vi "UMLEditor CreateNoteText.vi"(1 "graph":refnum<class "Graph.lvclass">, 2 "NoteEdge?":refnum<class "AbstractEdge.lvclass">, 5 "error in (no error)":errorcluster) -> (19 "error out":errorcluster)   [LabVIEW 2020]
doc: "Gets current diagram values"
uses:
  <resource>/Framework/Providers/Open_GDS/UML/Graph_class/Graph.lvclass
  <resource>/Framework/Providers/Open_GDS/UML/AbstractEdge_class/AbstractEdge.lvclass
  <resource>/Framework/Providers/Open_GDS/UML/General/Point/Point Point2D.ctl
  <resource>/Framework/Providers/Open_GDS/UML/NoteNode_class/NoteNode.lvclass
  <resource>/Framework/Providers/Open_GDS/UML/AbstractNode_class/AbstractNode.lvclass
  <resource>/Framework/Providers/Open_GDS/UML/MultiLineString_class/MultiLineString.lvclass
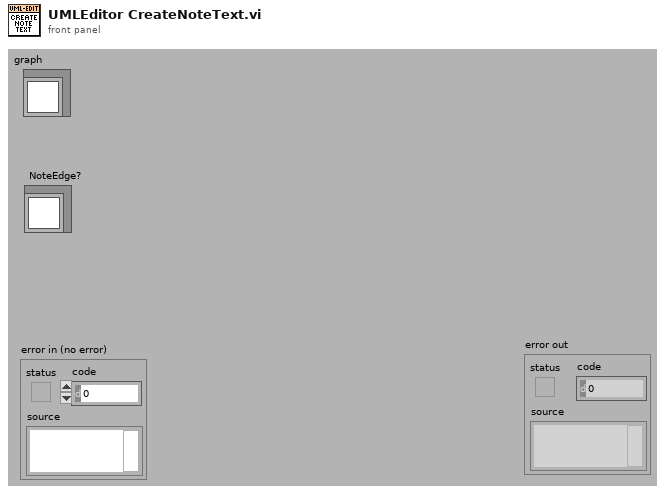
[diagram p1: front panel]
types:
  T1 = typedef "Point Point2D.ctl" = cluster{"x":dbl, "y":dbl}
  T2 = cluster{"text":string, "empty picture":picture, string}
  T3 = typedef "Rectangle Rectangle2D.ctl" = cluster{"x":dbl, "y":dbl, "width":dbl, "height":dbl}
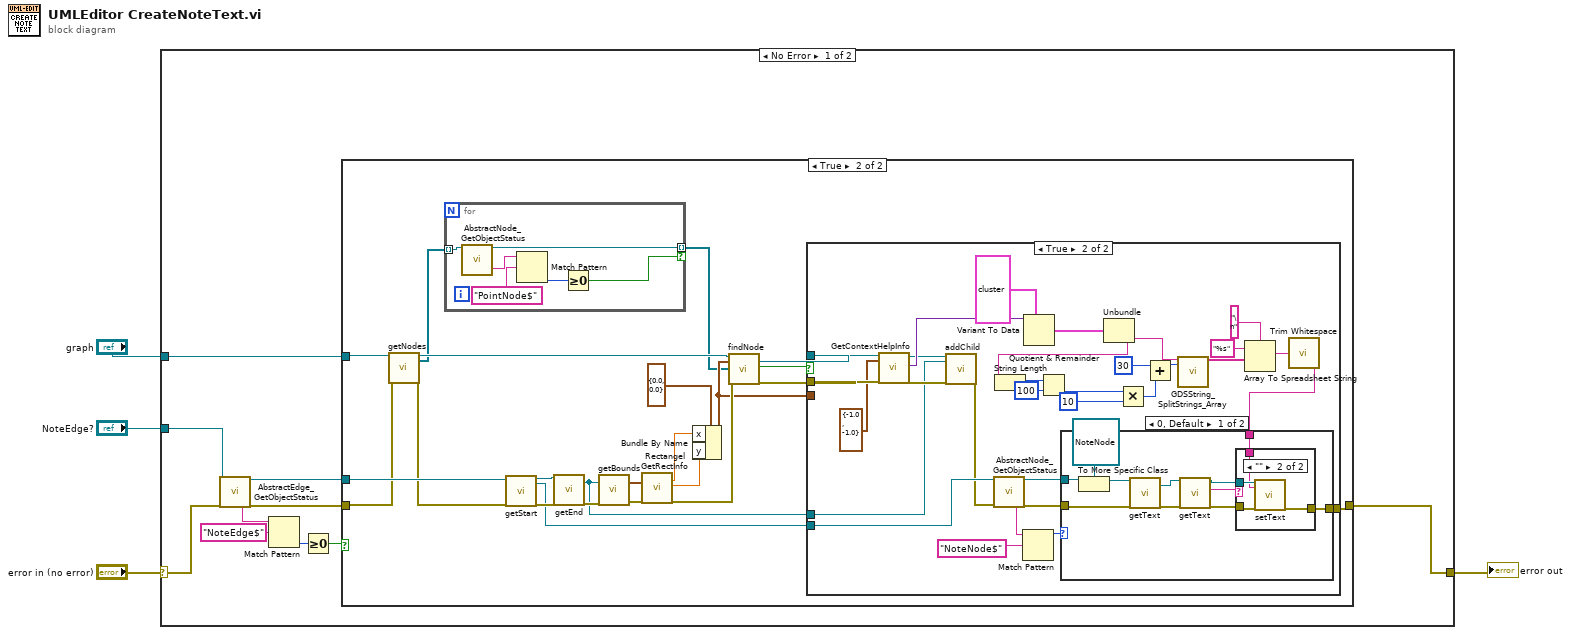
[diagram p0: block diagram]
diagram:
  n1 = case shown="No Error" "error in (no error)" {
    selector: "error in (no error)" -> [w8 w93]
    tunnel: [w7 w93] -> w3
    tunnel: "NoteEdge?" -> [w10 _]
    tunnel: "graph" -> [w6 _]
    frame No Error {
      n2 = call <resource>:"AbstractEdge_GetObjectStatus.vi"("reference in"=w10, "error in (no error)"=w8) -> ("Class name"=w13:string, "reference out"=w5:refnum<class "AbstractEdge.lvclass">, "error out"=w14:errorcluster)  [unwired: 9 in, 6 out]
      n3 = Match Pattern(string=w13, regular expression="NoteEdge$") -> (offset past match=w11:i32)  [unwired: 4 out]
      n4 = Greater Or Equal To 0?(x=w11) -> (x >= 0?=w9:bool)
      n5 = case shown="True" w9 {
        tunnel: w14 -> [w15 w25]
        tunnel: [w15 w20] -> w7
        tunnel: w6 -> [_ w27]
        tunnel: w5 -> [_ w37]
        frame False {
        }
        frame True {
          n6 = call-dynamic "getNodes.vi"("reference"=w27, "error in (no error)"=w25) -> ("reference out"=w26:refnum<class "Graph.lvclass">, "nodes"=w23:refnum<class "AbstractNode.lvclass">[], "error out"=w24:errorcluster)  [unwired: 15 in]
          n7 = for {
            tunnel: w23 -> [w42] mode=indexing
            tunnel: [w40] -> w16 mode=indexing if=w39
            n8 = call <resource>:"AbstractNode_GetObjectStatus.vi"("reference in"=w42) -> ("Class name"=w41:string, "reference out"=w40:refnum<class "AbstractNode.lvclass">)  [unwired: 1 in, 16 out]
            n9 = Match Pattern(string=w41, regular expression="PointNode$") -> (offset past match=w44:i32)  [unwired: 4 out]
            n10 = Greater Or Equal To 0?(x=w44) -> (x >= 0?=w39:bool)
          }
          n11 = call-dynamic "getStart.vi"("reference"=w37, "error in (no error)"=w24) -> ("reference out"=w36:refnum<class "AbstractEdge.lvclass">, "startNode"=w19:refnum<class "AbstractNode.lvclass">, "error out"=w38:errorcluster)  [unwired: 14 in, 1 out]
          n12 = call-dynamic "getEnd.vi"("reference"=w36, "error in (no error)"=w38) -> ("endNode"=w17:refnum<class "AbstractNode.lvclass">, "error out"=w35:errorcluster)  [unwired: 14 in, 2 out]
          n13 = call-dynamic "getBounds.vi"("reference"=w17, "error in (no error)"=w35) -> ("bounds"=w34:T3, "error out"=w33:errorcluster)  [unwired: 15 in, 1 out]
          n14 = call <resource>:"Rectangel GetRectInfo.vi"("bounds"=w34, "error in (no error)"=w33) -> ("centerX"=w22:dbl, "centerY"=w21:dbl, "error out"=w31:errorcluster)  [unwired: 15 out]
          n15 = Bundle By Name(cluster=T1 {"x"=0.0, "y"=0.0} ("point2D"), "x"=w22, "y"=w21) -> (w28:T1)
          n16 = call-dynamic "findNode.vi"("reference"=w26, "point2D"=w28, "IgnoreTheseNodes"=w16, "error in (no error)"=w31) -> ("node"=w30:refnum<class "AbstractNode.lvclass">, "found"=w18:bool, "error out"=w29:errorcluster)  [unwired: 12 in, 1 out]
          n17 = case shown="True" w18 {
            tunnel: w30 -> [_ w75]
            tunnel: w29 -> [w45 w74]
            tunnel: w28 -> [_ _]
            tunnel: [w45 w65] -> w20
            tunnel: w19 -> [_ w64]
            tunnel: w17 -> [_ w60]
            frame False {
            }
            frame True {
              n18 = call-dynamic "GetContextHelpInfo.vi"("reference"=w75, "MousePos"=T1 {"x"=-1.0, "y"=-1.0}, "error in (no error)"=w74) -> ("reference out"=w63:refnum<class "AbstractNode.lvclass">, "ContextHelpInfo"=w73:variant, "error out"=w62:errorcluster)  [unwired: 13 in, 1 out]
              n19 = call-dynamic "addChild.vi"("reference"=w63, "node"=w60, "error in (no error)"=w62) -> ("error out"=w61:errorcluster)  [unwired: 15 in, 1 out]
              n20 = call <resource>:"AbstractNode_GetObjectStatus.vi"("reference in"=w64, "error in (no error)"=w61) -> ("Class name"=w69:string, "reference out"=w66:refnum<class "AbstractNode.lvclass">, "error out"=w67:errorcluster)  [unwired: 15 out]
              n21 = Match Pattern(string=w69, regular expression="NoteNode$") -> (offset past match=w68:i32)  [unwired: 4 out]
              n22 = Variant To Data(type=T2 {"text"="", "empty picture"=bytes[0], ""} ("output cluster"), Variant=w73) -> (data=w71:T2)  [unwired: 1 in, 1 out]
              n23 = Unbundle(w71) -> (w54:string)  [unwired: 2 out]
              n24 = String Length(string=w54) -> (length=w53:i32)
              n25 = Quotient & Remainder(x=w53, y=100) -> (floor(x/y)=w49:i32)  [unwired: 1 out]
              n26 = Multiply(x=w49, y=10) -> (x*y=w47:i32)
              n27 = Add(x=30, y=w47) -> (x+y=w51:i32)
              n28 = call <resource>:"GDSString_SplitStrings_Array.vi"("string"=w54, "Max string length"=w51) -> ("Array"=w59:string[])  [unwired: 17 out]
              n29 = Array To Spreadsheet String(delimiter (Tab)="\n", array=w59, 3:"%s" ("format string")) -> (spreadsheet string=w56:string)
              n30 = call <vilib>:"Trim Whitespace.vi"("string"=w56) -> ("trimmed string"=w55:string)  [unwired: 1 in]
              n31 = case shown="0, Default" w68 {
                tunnel: w67 -> [w86 w92]
                tunnel: w66 -> [w77 _]
                tunnel: [w81 w92] -> w65
                tunnel: w55 -> [w80 _]
                frame 0, Default {
                  n32 = To More Specific Class(target class=refnum<class "NoteNode.lvclass"> refnum ("reference"), reference=w77) -> (specific class reference=w76:refnum<class "NoteNode.lvclass">)  [unwired: 1 in, 1 out]
                  n33 = call-dynamic "getText.vi"("reference"=w76, "error in (no error)"=w86) -> ("text"=w79:refnum<class "MultiLineString.lvclass">, "error out"=w85:errorcluster)  [unwired: 15 in, 1 out]
                  n34 = call-dynamic "getText.vi"("reference"=w79, "error in (no error)"=w85) -> ("reference out"=w82:refnum<class "MultiLineString.lvclass">, "text"=w84:string, "error out"=w83:errorcluster)  [unwired: 15 in]
                  n35 = case shown="\"\"" w84 {
                    tunnel: w83 -> [w87 w91]
                    tunnel: w82 -> [_ w90]
                    tunnel: [w87 w89] -> w81
                    tunnel: w80 -> [_ w88]
                    frame "False", Default {
                    }
                    frame "" {
                      n36 = call-dynamic "setText.vi"("reference"=w90, "text"=w88, "error in (no error)"=w91) -> ("error out"=w89:errorcluster)  [unwired: 15 in, 1 out]
                    }
                  }
                }
                frame -1 {
                }
              }
            }
          }
        }
      }
    }
    frame Error {
    }
  }
  "error out" <- w3
